vi "Create Type Definitions.vi"(11 "Test Case In":refnum<class "Runner Unit Test - Create Files.lvclass">) -> (0 "error out":errorcluster, 3 "Test Case Out":refnum<class "Runner Unit Test - Create Files.lvclass">)   [LabVIEW 2026, in "Runner Unit Test - Create Files.lvclass"]
uses:
  Runner Unit Test - Create Files.lvclass
  C:/Program Files/National Instruments/LabVIEW 2026/vi.lib/Astemes/LUnit/Test Case.lvclass
  Actors/Runner/Runner/Runner.lvclass
  Interfaces/IRunner/IRunner/Interfaces--cluster.ctl
  Interfaces/IProject Manager/IProject Manager.lvclass
  Interfaces/IFile Manager/IFile Manager.lvclass
  Interfaces/IPython Caller/IPython Caller.lvclass
  Interfaces/IElement Manager/IElement Manager.lvclass
  Interfaces/ILV File Creator/ILV File Creator.lvclass
  Interfaces/IHash Whitelist Handler/IHash Whitelist Handler.lvclass
  Actors/Mock Logger/Mock Logger/Mock Logger.lvclass
  C:/Program Files/National Instruments/LabVIEW 2026/vi.lib/ActorFramework/Actor/Actor.lvclass
  Type Definitions/Analysis Output--cluster.ctl
  Type Definitions/Type Definition--cluster.ctl
  Type Definitions/Parameter--cluster.ctl
  Type Definitions/Function--cluster.ctl
  <vilib>/ActorFramework/Message Enqueuer/Message Enqueuer.lvclass/Message Enqueuer.ctl
  <vilib>/ActorFramework/Message Enqueuer/Enqueue.vi
  Mocks/Mock IFile Manager/Mock IFile Manager.lvclass
  C:/Program Files/National Instruments/LabVIEW 2026/vi.lib/Astemes/LMock/Mock.lvclass
  C:/Users/juanj/Documents/hasbun_wood_engineering/github/py2vi/labview/Interfaces/IFile Manager/IFile Manager.lvclass
  Mocks/Mock IPython Caller/Mock IPython Caller.lvclass
  C:/Users/juanj/Documents/hasbun_wood_engineering/github/py2vi/labview/Interfaces/IPython Caller/IPython Caller.lvclass
  <vilib>/ActorFramework/Stop Msg/Stop Msg.lvclass
  C:/Program Files/National Instruments/LabVIEW 2026/vi.lib/ActorFramework/Message/Message.lvclass
  <vilib>/Astemes/LMock/Exactly Identical Inputs.vi
  <vilib>/ActorFramework/Message Priority Queue/Priority Enqueue.vi
  Runner Unit Test - Create Files.lvclass/Runner Unit Test - Create Files.ctl
  C:/Users/juanj/Documents/hasbun_wood_engineering/github/py2vi/labview/Mocks/Mock IFile Manager/Mock IFile Manager.lvclass
  Interfaces/IRunner/IRunner/IRunner.lvclass
  <vilib>/ActorFramework/Actor/Actor.lvclass
  <vilib>/Astemes/LMock/LMock Verifier.lvclass
  <vilib>/Astemes/LMock/LMock.lvlib
  <vilib>/Astemes/LMock/LMock Exactly.lvlib
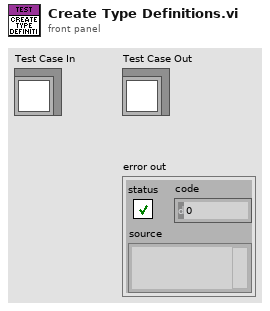
[diagram p1: front panel]
types:
  T1 = typedef "Function--cluster.ctl" = cluster{"name":string, "docstring":string, "input_parameters":T2[], "output_parameters":T2[]}
  T2 = typedef "Parameter--cluster.ctl" = cluster{"name":string, "data_type":string, "container":string, "dimensions":i32, "type_definition":string}
  T3 = typedef "Type Definition--cluster.ctl" = cluster{"name":string, "fields":T2[]}
  T4 = typedef "Analysis Output--cluster.ctl" = cluster{"type_definitions":T3[], "functions":T1[]}
  T5 = typedef "IRunner.lvlib/IRunner.lvclass/Interfaces--cluster.ctl" = cluster{"IProject Manager":refnum<class "IProject Manager.lvclass">, "IFile Manager":refnum<class "IFile Manager.lvclass">, "IPython Caller":refnum<class "IPython Caller.lvclass">, "IElement Manager":refnum<class "IElement Manager.lvclass">, "ILV File Creator":refnum<class "ILV File Creator.lvclass">, "IHash Whitelist Handler":refnum<class "IHash Whitelist Handler.lvclass">}
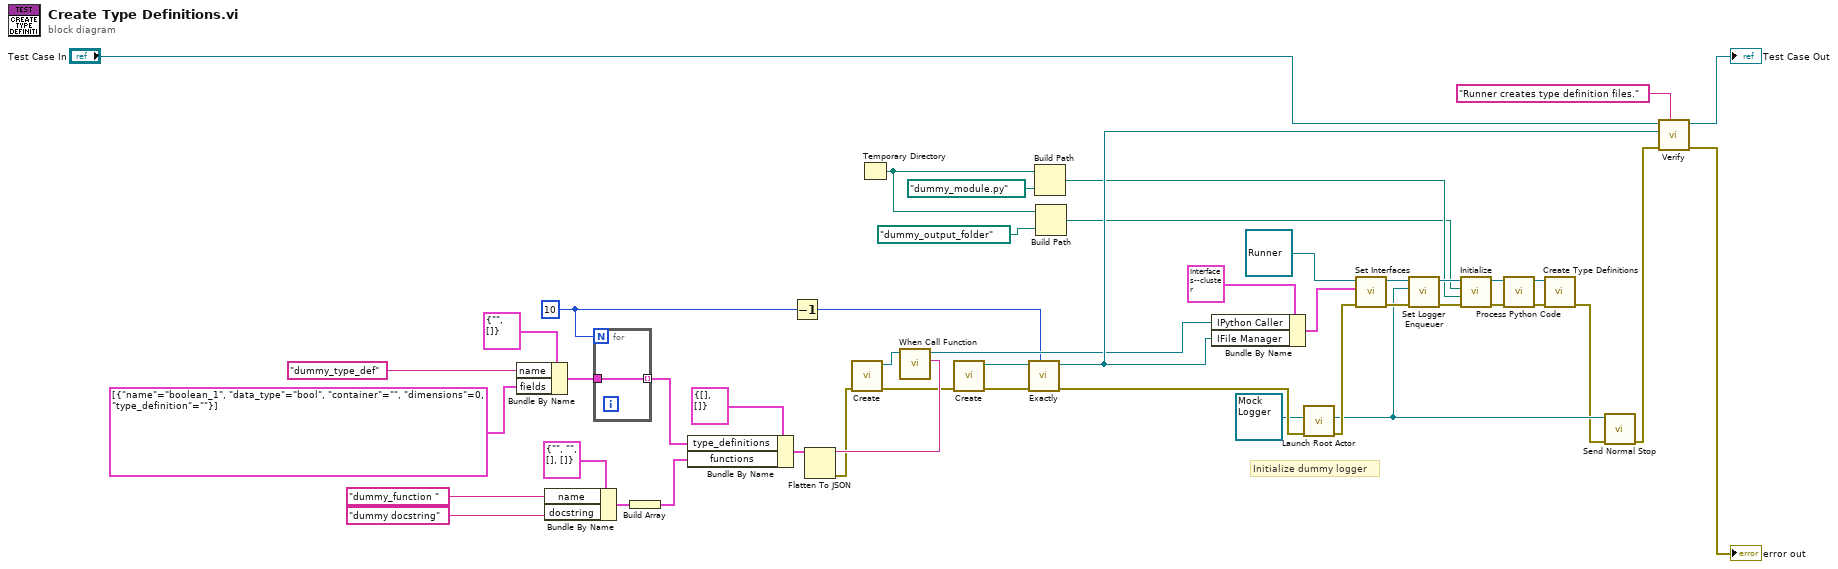
[diagram p0: block diagram]
diagram:
  w10 = 10
  # "Initialize dummy logger"
  n1 = Bundle By Name(cluster=T3 {"name"="", "fields"=[]} ("Type Definition"), "name"="dummy_type_def", "fields"=T2[] [{"name"="boolean_1", "data_type"="bool", "container"="", "dimensions"=0, "type_definition"=""}]) -> (w13:T3)
  n2 = Bundle By Name(cluster=T1 {"name"="", "docstring"="", "input_parameters"=[], "output_parameters"=[]} ("Function"), "name"="dummy_function ", "docstring"="dummy docstring") -> (w16:T1)
  n3 = for {
    N: w10 -> [_]
    tunnel: w13 -> [w49]
    tunnel: [w49] -> w12 mode=indexing
  }
  n4 = Build Array(w16) -> (w15:T1[])
  n5 = Bundle By Name(cluster=T4 {"type_definitions"=[], "functions"=[]} ("Analysis Output"), "type_definitions"=w12, "functions"=w15) -> (w14:T4)
  n6 = Decrement(x=w10) -> (x-1=w1:i32)
  n7 = Flatten To JSON(anything=w14) -> (JSON string=w11:string, 11:w7:errorcluster)  [unwired: 2 in]
  n8 = call "Create.vi"("error in (no error)"=w7) -> ("error out"=w9:errorcluster, "Mock Class Generator out"=w24:refnum<class "Mock IPython Caller.lvclass">)  [unwired: 9 in]
  n9 = Temporary Directory() -> (w32:path)
  n10 = call "When Call Function.vi"("Return String"=w11, "IPython Caller in"=w24) -> ("IPython Caller out"=w8:refnum<class "Mock IPython Caller.lvclass">)  [unwired: 9 in]
  n11 = call "Create.vi"("error in (no error)"=w9) -> ("error out"=w47:errorcluster, "Mock Class Generator out"=w38:refnum<class "Mock IFile Manager.lvclass">)  [unwired: 9 in]
  n12 = call-poly <vilib>:"Exactly.vi"("Expected Number of Calls"=w1, "error in (no error)"=w47, "Mock in"=w38) -> ("error out"=w46:errorcluster, "Mock out"=w37:refnum<class "Mock IFile Manager.lvclass">)  [unwired: 7 in]
  n13 = Build Path(base path=w32, name or relative path=path "dummy_module.py") -> (appended path=w29:path)
  n14 = Build Path(base path=w32, name or relative path=path "dummy_output_folder") -> (appended path=w28:path)
  n15 = Bundle By Name(cluster=T5 {"IProject Manager"=refnum, "IFile Manager"=refnum, "IPython Caller"=refnum, "IElement Manager"=refnum, "ILV File Creator"=refnum, "IHash Whitelist Handler"=refnum} ("Interfaces"), "IPython Caller"=w8, "IFile Manager"=w37) -> (w39:T5)
  n16 = call <vilib>:"Launch Root Actor.vi"("error in (no error)"=w46, "Actor"=refnum<class "Mock Logger.lvclass"> refnum ("Mock Logger.lvlib:Mock Logger.lvclass")) -> ("error out"=w45:errorcluster, "Actor's Enqueuer"=w35:refnum<class "Message Enqueuer.lvclass">)  [unwired: 8 in]
  n17 = call-dynamic "Set Interfaces.vi"("error in"=w45, "Interfaces"=w39, "Runner in"=refnum<class "Runner.lvclass"> refnum ("Runner.lvlib:Runner.lvclass")) -> ("error out"=w48:errorcluster, "Runner out"=w41:refnum<class "Runner.lvclass">)  [unwired: 7 in]
  n18 = call-dynamic "Set Logger Enqueuer.vi"("error in"=w48, "Logger"=w35, "Runner in"=w41) -> ("error out"=w43:errorcluster, "Runner out"=w33:refnum<class "Runner.lvclass">)  [unwired: 7 in]
  n19 = call-dynamic "Initialize.vi"("error in"=w43, "Python Module"=w29, "Output Folder"=w28, "G-CLI Runner in"=w33) -> ("error out"=w4:errorcluster, "G-CLI Runner out"=w6:refnum<class "Runner.lvclass">)  [unwired: 6 in]
  n20 = call-dynamic "Process Python Code.vi"("error in"=w4, "G-CLI Runner in"=w6) -> ("error out"=w3:errorcluster, "G-CLI Runner out"=w5:refnum<class "Runner.lvclass">)  [unwired: 8 in]
  n21 = call-dynamic "Create Type Definitions.vi"("error in"=w3, "Runner in"=w5) -> ("error out"=w2:errorcluster)  [unwired: 8 in, 1 out]
  n22 = call <vilib>:"Send Normal Stop.vi"("error in (no error)"=w2, "Message Enqueuer"=w35) -> ("error out"=w44:errorcluster)  [unwired: 9 in]
  n23 = call <vilib>:"Verify.vi"("Description"="Runner creates type definition files.", "error in (no error)"=w44, "Mock"=w37, "LUnit Test Case In"="Test Case In") -> ("error out"=→"error out":errorcluster, "LUnit Test Case Out"=→"Test Case Out":refnum<class "Runner Unit Test - Create Files.lvclass">)  [unwired: 6 in]
